vi "Make Config.vi"(9 "Port Configuration":T7={"Mode"=enum."CAN FD", "Baud Rate"=500000, "Temination On"=TRUE, "Subordinate"=FALSE, "Echo TX"=FALSE, "FD Config"={"FD Baud Rate"=2000000, "ISO Mode"=TRUE, "BRS Enabled"=TRUE}} {"FD Config"."FD Baud Rate" format="%.0p"; "Baud Rate" format="%.0p"}, 10 "channel":u8, 11 "host":string) -> (3 "config":T1={"connection"={"host"="", "channel"=2, "cert path"=path "/home/lvuser/cansub_root_cert.crt"}, "bit rates"={"nominal bit rate"=500000, "nominal sample point"=80.0, "data bit rate"=2000000, "data sample point"=80.0}, "listen only"=FALSE, "filters"=[], "read mode"=enum."Poll", "max bytes per read"=4096, "reader FIFO depth"=0, "reader priority"=0, "ownership"=enum."Direct"} {"filters"."f2" format="%.0x"; "filters"."f1" format="%.0x"})   [LabVIEW 2021, in "CAN RW CANsub.lvclass"]
uses:
  CAN RW CANsub.lvclass
  <vilib>/CIF Foundation/CIF CAN RW Core/typedef/CAN Mode.ctl
  <vilib>/CIF Foundation/CIF CAN RW Core/CAN_RW_CORE.lvclass
  CANsub/common/Typedefs/CANsub_connection.ctl
  CANsub/common/CANsub_Common.lvlib
  CANsub/common/Typedefs/CANsub_Bit_Rates.ctl
  CANsub/c_client/api/Typedefs/CANsub_Filter.ctl
  CANsub/c_client/api/CANsub_API.lvlib
  CANsub/c_client/api/Typedefs/CANsub_Read_Mode.ctl
  CANsub/c_client/api/Typedefs/CANsub_Ownership.ctl
  CANsub/c_client/api/Typedefs/CANsub_Config.ctl
  <vilib>/CIF Foundation/CIF CAN RW Core/typedef/FD Config.ctl
  <vilib>/CIF Foundation/CIF CAN RW Core/typedef/CAN Port Configuration.ctl
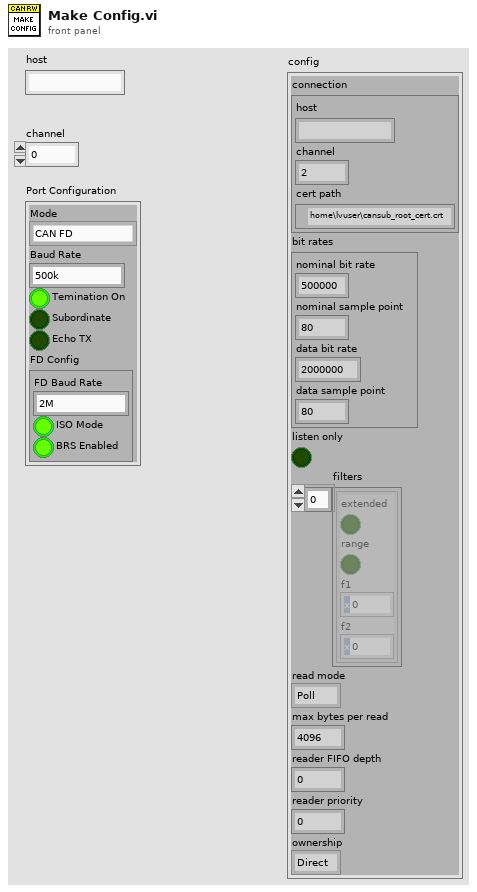
[diagram p1: front panel]
types:
  T1 = typedef "CANsub_API.lvlib/CANsub_Config.ctl" = cluster{"connection":T2, "bit rates":T3, "listen only":bool, "filters":T4[], "read mode":T5, "max bytes per read":i32, "reader FIFO depth":i32, "reader priority":i32, "ownership":T6}
  T2 = typedef "CANsub_Common.lvlib/CANsub_connection.ctl" = cluster{"host":string, "channel":u8, "cert path":path}
  T3 = typedef "CANsub_Common.lvlib/CANsub_Bit_Rates.ctl" = cluster{"nominal bit rate":u32, "nominal sample point":dbl, "data bit rate":u32, "data sample point":dbl}
  T4 = typedef "CANsub_API.lvlib/CANsub_Filter.ctl" = cluster{"extended":bool, "range":bool, "f1":u32, "f2":u32}
  T5 = typedef "CANsub_API.lvlib/CANsub_Read_Mode.ctl" = enum16{"Poll", "Reader"}
  T6 = typedef "CANsub_API.lvlib/CANsub_Ownership.ctl" = enum16{"Direct", "Shared"}
  T7 = typedef "CAN_RW_CORE.lvclass/CAN Port Configuration.ctl" = cluster{"Mode":T8, "Baud Rate":u64, "Temination On":bool, "Subordinate":bool, "Echo TX":bool, "FD Config":T9}
  T8 = typedef "CAN_RW_CORE.lvclass/CAN Mode.ctl" = enum16{"CAN 2.0", "CAN FD"}
  T9 = typedef "CAN_RW_CORE.lvclass/FD Config.ctl" = cluster{"FD Baud Rate":u64, "ISO Mode":bool, "BRS Enabled":bool}
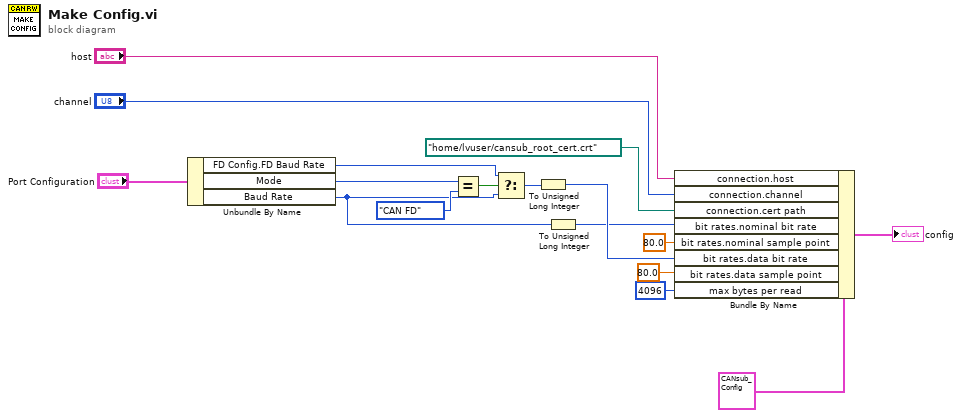
[diagram p0: block diagram]
diagram:
  n1 = Unbundle By Name("Port Configuration") -> ("FD Config.FD Baud Rate"=w13:u64, "Mode"=w16:T8, "Baud Rate"=w12:u64)
  n2 = Equal?(x=w16, y=CAN_Mode."CAN FD" ("Mode")) -> (x = y?=w14:bool)
  n3 = Select(t=w13, s=w14, f=w12) -> (s? t:f=w11:u64)
  n4 = To Unsigned Long Integer(number=w11) -> (unsigned 32bit integer=w7:u32)
  n5 = To Unsigned Long Integer(number=w12) -> (unsigned 32bit integer=w5:u32)
  n6 = Bundle By Name(cluster=T1 {"connection"={"host"="", "channel"=2, "cert path"=path "/home/lvuser/cansub_root_cert.crt"}, "bit rates"={"nominal bit rate"=500000, "nominal sample point"=80.0, "data bit rate"=2000000, "data sample point"=80.0}, "listen only"=FALSE, "filters"=[], "read mode"=enum."Poll", "max bytes per read"=4096, "reader FIFO depth"=0, "reader priority"=0, "ownership"=enum."Direct"} ("CANsub_Config"), "connection.host"="host", "connection.channel"="channel", "connection.cert path"=path "/home/lvuser/cansub_root_cert.crt", "bit rates.nominal bit rate"=w5, "bit rates.nominal sample point"=80.0, "bit rates.data bit rate"=w7, "bit rates.data sample point"=80.0, "max bytes per read"=4096) -> (→"config":T1)
